vi "07-get-and_display_image.vi"() -> ()   [LabVIEW 2018, in "LV2Julia_examples.lvlib"]
uses:
  LV2Julia_examples.lvlib
  LV2Julia_core/VIs/Server or client state.ctl
  LV2Julia_core/VIs/Commands.ctl
  c965f866-6df0-488f-ad0f-a92a8fae8aa7.vi
  f9264f0d-2c2d-4a22-a0da-9e005a3dfb77.vi
  c965f866-6df0-488f-ad0f-a92a8fae8aa7.vi/33124eee-61ee-47ce-a2ee-a316e75573f0.vi
  f9264f0d-2c2d-4a22-a0da-9e005a3dfb77.vi/2e383da5-81e8-4d2f-838e-0096a58cac2b.vi
  c965f866-6df0-488f-ad0f-a92a8fae8aa7.vi/33124eee-61ee-47ce-a2ee-a316e75573f0.vi/d68d7647-4093-4c43-ac50-45e8617a67d4.vi
  c965f866-6df0-488f-ad0f-a92a8fae8aa7.vi/33124eee-61ee-47ce-a2ee-a316e75573f0.vi/d4dd76be-dac1-4fb1-9b61-ff498888781d.vi
  c965f866-6df0-488f-ad0f-a92a8fae8aa7.vi/33124eee-61ee-47ce-a2ee-a316e75573f0.vi/3d2936eb-e328-4fb1-a033-36a2eec84a7e.vi
  f9264f0d-2c2d-4a22-a0da-9e005a3dfb77.vi/2e383da5-81e8-4d2f-838e-0096a58cac2b.vi/a5eb823d-2e81-433a-a2a4-d72f4d0f5ad1.vi
  f9264f0d-2c2d-4a22-a0da-9e005a3dfb77.vi/2e383da5-81e8-4d2f-838e-0096a58cac2b.vi/4dce512e-2117-4d69-9680-b4170fc60420.vi
  f9264f0d-2c2d-4a22-a0da-9e005a3dfb77.vi/2e383da5-81e8-4d2f-838e-0096a58cac2b.vi/a0e64533-fd0c-487f-a6cc-44784a851655.vi
  LV2Julia_core/VIs/check ID validity.vi
  LV2Julia_core/VIs/bindata_descr to JSON.vi
  LV2Julia_core/VIs/check cluster field names.vi
  LV2Julia_core/VIs/concat JSON.vi
  LV2Julia_core/VIs/build request.vi
  LV2Julia_core/VIs/Parse server response.vi
  LV2Julia_core/VIs/log jl exceptions.vi
  LV2Julia_core/VIs/jl-scripts path.vi
  LV2Julia_core/LV2Julia_core.lvlib
panel:
  out "img_type":string
  out "picture":picture
  in  "select image":u16(ring) items=["airplaneF16.tiff", "autumn_leaves.png", "barbara_color.png", "barbara_gray_512.bmp", "blobs.gif", "cameraman.tif", "chelsea.png", "coffee.png", "earth_apollo17.jpg", "fabio_color_256.png", "fabio_color_512.png", "fabio_gray_256.png", "fabio_gray_512.png", "hela-cells.tif", "house.tif", "jetplane.tif", "lake_color.tif", "lake_gray.tif", "lena_color_256.tif", "lena_color_512.tif", "lena_gray_256.tif", "lena_gray_512.tif", "lena_gray_16bit.png", "livingroom.tif", "lighthouse.png", "mandril_color.tif", "mandril_gray.tif", "mandrill.tiff", "m51.tif", "monarch_color.png", "monarch_color_256.png", "moonsurface.tiff", "morphology_test_512.tiff", "mountainstream.png", "peppers_color.tif", "peppers_gray.tif", "pirate.tif", "resolution_test_512.tif", "resolution_test_1920.tif", "sudoku.tiff", "toucan.png", "walkbridge.tif", "woman_blonde.tif", "woman_darkhair.tif"]
  out "short error info":string
  in  "next":bool
  out "current error":errorcluster
  out "final error":errorcluster
  in  "stop":bool
  out "ZMQ timeout":bool
  out "Julia script file path":path
  out "temporary script path":path
  out "Jl Server state":T1
  # "using TestImages, ImageMagick"
  # "If you don't see any received picture in this pane. check the scrollbars!"
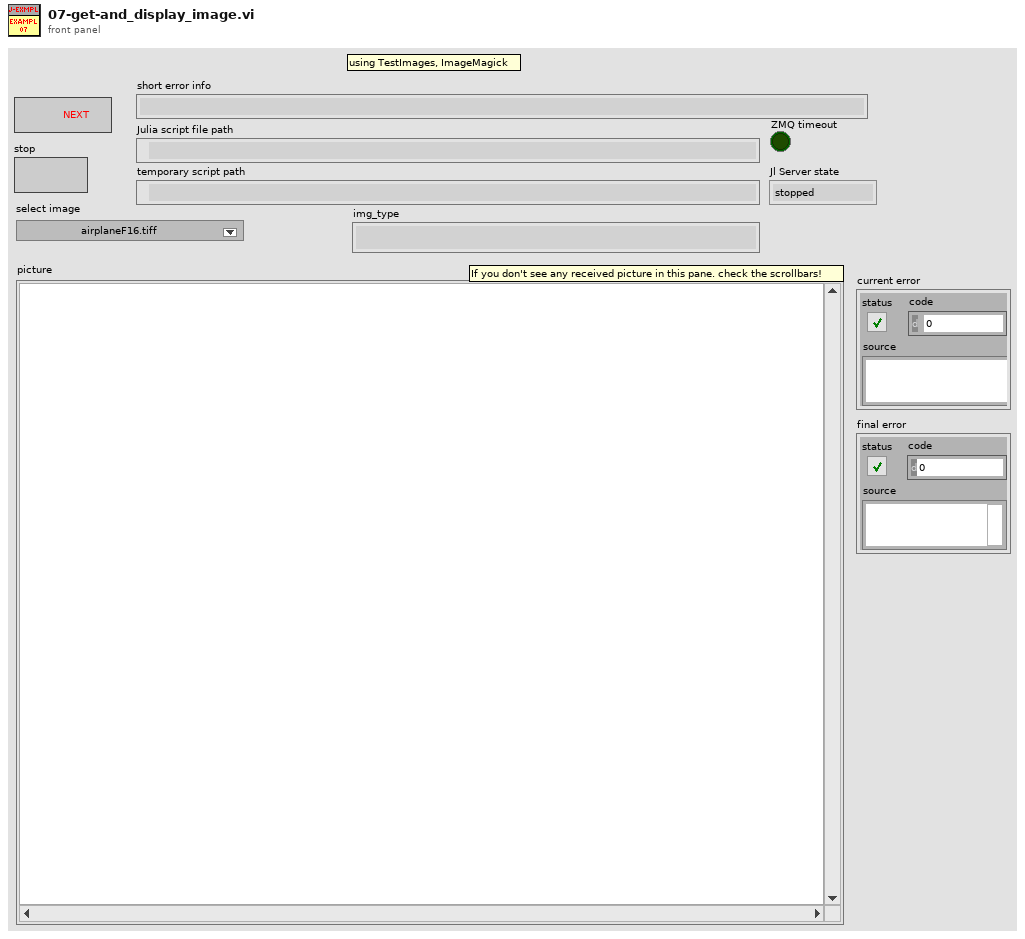
[diagram p1: front panel]
types:
  T1 = typedef "LV2Julia_core.lvlib/Server or client state.ctl" = enum16{"stopped", "running", "unknown"}
  T2 = typedef "LV2Julia_core.lvlib/Commands.ctl" = enum16{"Start Jl-server & Init LV-client", "Send request & Get response ", "Stop Jl-server & Cleanup LV-client", "Cleanup LV-client", "Start Jl-server", "Stop Jl-server", "Init LV-Client", "Cleanup LV-Client", "(not allowed)", "Set LV Client state", "Set Jl Server state", "set ZMQ timeout", "read ZMQ timeout", "read-out state"}
  T3 = typedef "LV2Julia_core.lvlib/detailed error info.ctl" = cluster{"exception_or_info":string, "trace":T4[]}
  T4 = typedef "LV2Julia_core.lvlib/StackFrame.ctl" = cluster{"frame_summary":string, "func":string, "linfo":string, "file":string, "line":i32, "pointer":u64, "from_c":bool, "inlined":bool}
  T5 = typedef "imagedata.ctl" = cluster{"image type":i32, "image depth":i32, "image":u8[], "mask":u8[], "colors":u32[], "Rectangle":cluster{"left":i16, "top":i16, "right":i16, "bottom":i16}}
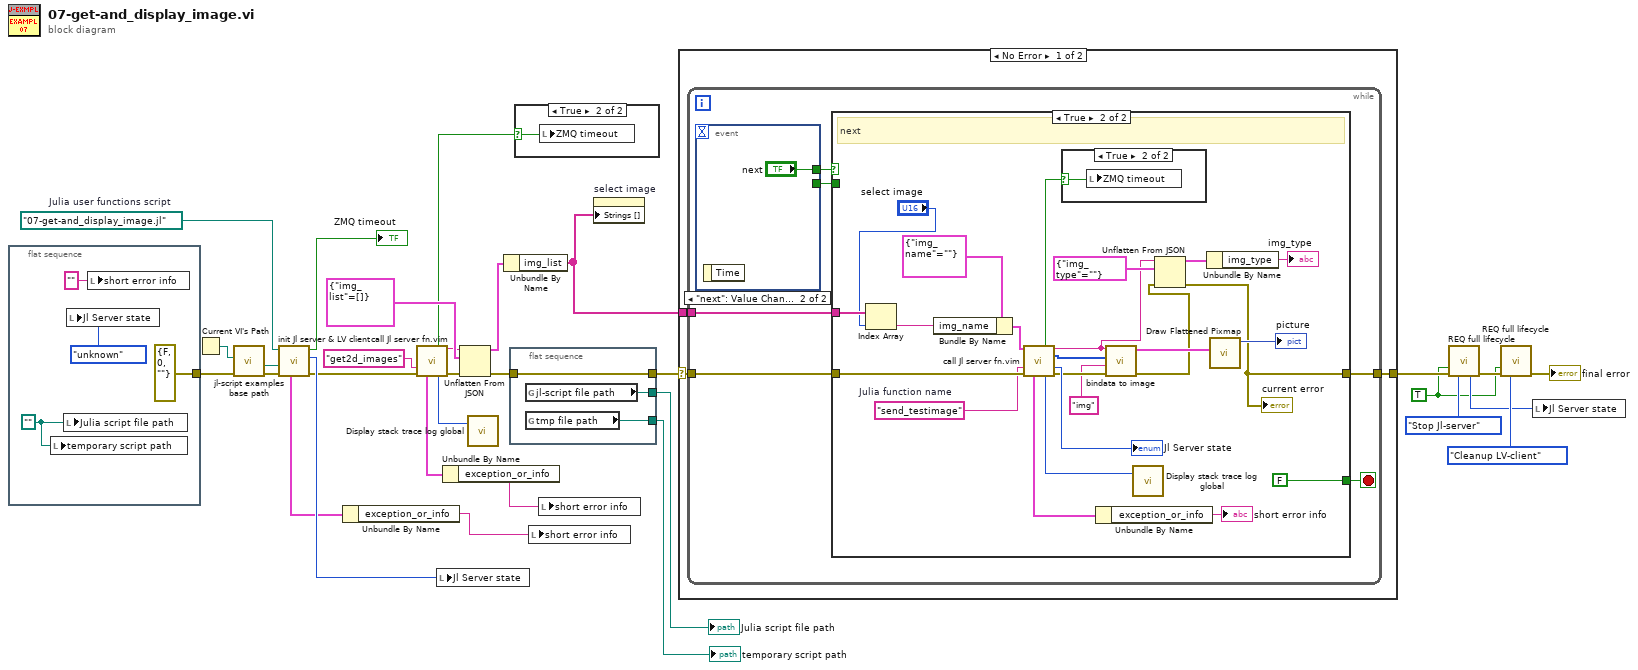
[diagram p0: block diagram]
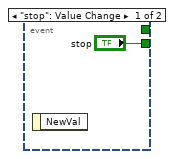
[diagram p3: hidden frame]
diagram:
  w10 = path "07-get-and_display_image.jl"  # Julia user functions script
  w22 = TRUE ("Force command")
  n1 = flat-sequence {
    tunnel: [errorcluster {"status"=FALSE, "code"=0, "source"=""} ("error in (no error)")] -> w4
    frame #0 {
      w33 = path ""
      n2 = local write "temporary script path"(w33) -> ()
      n3 = local write "Julia script file path"(w33) -> ()
      n4 = local write "Jl Server state"(Server_or_client_state."unknown" ("Jl Server state out")) -> ()
      n5 = local write "short error info"("" ("short error info")) -> ()
    }
  }
  n6 = Current VI's Path() -> (path=w6:path)
  n7 = call "jl-script examples base path.vi"("error in (no error)"=w4, "calling example VI path"=w6) -> ("error out"=w5:errorcluster, "jl-script-examples base path"=w3:path)  [unwired: 8 in]
  n8 = call "init Jl server & LV client.vi"("error in (no error)"=w5, "Base path (not a path)"=w3, "Julia user functions script"=w10) -> ("error out"=w7:errorcluster, "Jl Server state out"=w8:T1, "timeout?"=→"ZMQ timeout":bool, "detailed error info"=w2:T3)  [unwired: 3 in, 2 out]
  n9 = Unbundle By Name(w2) -> ("exception_or_info"=w1:string)
  n10 = call "call Jl server fn.vim"("fun2call"="get2d_images", "error in (no error)"=w7) -> ("timeout?"=w15:bool, "JSON received"=w17:string, "detailed error info"=w14:T3, "return code"=w12:u8, "error out"=w16:errorcluster)  [unwired: 7 in, 2 out]
  n11 = local write "Jl Server state"(w8) -> ()
  n12 = Unbundle By Name(w14) -> ("exception_or_info"=w13:string)
  n13 = Unflatten From JSON(JSON string=w17, type and defaults=cluster{"img_list":string[]} {"img_list"=[]} ("parsed response"), error in (no error)=w16) -> (value=w19:cluster{"img_list":string[]}, error out=w21:errorcluster)  [unwired: 4 in]
  n14 = call "Display stack trace log global.vi"("server return code"=w12) -> ()  [unwired: 3 in]
  n15 = Unbundle By Name(w19) -> ("img_list"=w11:string[])
  n16 = flat-sequence {
    tunnel: [w38] -> w26
    tunnel: w21 -> [w38]
    tunnel: [w37] -> w24
    tunnel: [w36] -> w25
    frame #0 {
      n17 = global read "jl-scripts path.vi" "jl-script file path"() -> (w37:path)
      n18 = global read "jl-scripts path.vi" "tmp file path"() -> (w36:path)
    }
  }
  n19 = case shown="True" w15 {
    selector: w15 -> [_ w39]
    frame False {
    }
    frame True {
      n20 = local write "ZMQ timeout"(w39) -> ()
    }
  }
  n21 = local write "short error info"(w1) -> ()
  n22 = local write "short error info"(w13) -> ()
  n23 = property on="select image" class="Ring (strict)"("Strings []"=w11) -> ()  [unwired: 2 in, 2 out]
  n24 = case shown="No Error" w26 {
    selector: w26 -> [w41 w78]
    tunnel: [w42 w78] -> w31
    tunnel: w11 -> [w40 _]
    frame No Error {
      n25 = while {
        tunnel: w41 -> [w47]
        tunnel: [w48] -> w42
        tunnel: w40 -> [w43]
        stop <- w45 stop-if-true
        n26 = event shown="[1] \"next\": Value Change" {
          selector: _ -> [_ _]
          dyn-events: _ -> [_ _]
          timeout: _ -> [_ _]
          tunnel: [_ "next"] -> w46
          tunnel: ["stop" _] -> w44
          event "stop": Value Change {
            n27 = event-data() -> ()  [unwired: 1 in, 1 out]
          }
          event "next": Value Change {
            n28 = event-data() -> ()  [unwired: 1 in, 1 out]
          }
        }
        n29 = case shown="True" w46 {
          tunnel: [w52 w54] -> w48
          tunnel: w47 -> [w52 w75]
          tunnel: [w51 FALSE ("stop this VI only")] -> w45
          tunnel: w44 -> [w51 _]
          tunnel: w43 -> [_ w66]
          frame False {
            # "stop"
          }
          frame True {
            w74 = "send_testimage"  # Julia function name
            # "next"
            n30 = Index Array(array=w66, index="select image") -> (element=w67:string)
            n31 = Bundle By Name(cluster=cluster{"img_name":string} {"img_name"=""} ("parsed response"), "img_name"=w67) -> (w64:cluster{"img_name":string})
            n32 = call "call Jl server fn.vim"("Arguments 1"=w64, "fun2call"=w74, "error in (no error)"=w75) -> ("timeout?"=w72:bool, "JSON received"=w53:string, "binary data received"=w60:u8[], "Jl Server state out"=→"Jl Server state":T1, "detailed error info"=w70:T3, "return code"=w71:u8, "error out"=w61:errorcluster)  [unwired: 6 in]
            n33 = case shown="True" w72 {
              selector: w72 -> [_ w77]
              frame False {
              }
              frame True {
                n34 = local write "ZMQ timeout"(w77) -> ()
              }
            }
            n35 = Unbundle By Name(w70) -> ("exception_or_info"=→"short error info":string)
            n36 = call "bindata to image.vi"("error in (no error)"=w61, "name"="img", "binary data in"=w60, "JSON in"=w53) -> ("error out"=w55:errorcluster, "img out"=w62:T5)  [unwired: 6 in]
            n37 = call "Display stack trace log global.vi"("server return code"=w71) -> ()  [unwired: 3 in]
            n38 = Unflatten From JSON(JSON string=w53, type and defaults=cluster{"img_type":string} {"img_type"=""}, error in (no error)=w55) -> (value=w57:cluster{"img_type":string}, error out=w54:errorcluster)  [unwired: 4 in]
            "current error" <- w54
            n39 = Unbundle By Name(w57) -> ("img_type"=→"img_type":string)
            n40 = call <vilib>:"Draw Flattened Pixmap.vi"("image data"=w62) -> ("new picture"=→"picture":picture)  [unwired: 8 in]
          }
        }
      }
    }
    frame Error {
    }
  }
  n41 = call "REQ full lifecycle.vi"("Force command"=w22, "error in"=w31, "command"=Commands."Stop Jl-server") -> ("Jl Server state out"=w23:T1, "error out"=w29:errorcluster)  [unwired: 6 in, 5 out]
  n42 = call "REQ full lifecycle.vi"("Force command"=w22, "error in"=w29, "command"=Commands."Cleanup LV-client") -> ("error out"=→"final error":errorcluster)  [unwired: 6 in, 6 out]
  n43 = local write "Jl Server state"(w23) -> ()
  "temporary script path" <- w25
  "Julia script file path" <- w24
